vi "Sell Stock.vi"(8 "error in":errorcluster, 10 "quantity":i32=1, 11 "Stock Name":string) -> (0 "error out":errorcluster, 3 "Order":T1)   [LabVIEW 2020, in "Full Featured MCP Server.lvlib"]
doc: "Sells shares of one stock at the current price and returns what was sold: stock, quantity, price per share, total and the wallet afterwards. The order is refused with an error that says why when the name is unknown or you own fewer shares than you want to sell."
uses:
  Full Featured MCP Server.lvlib
  Market/Market Mode.ctl
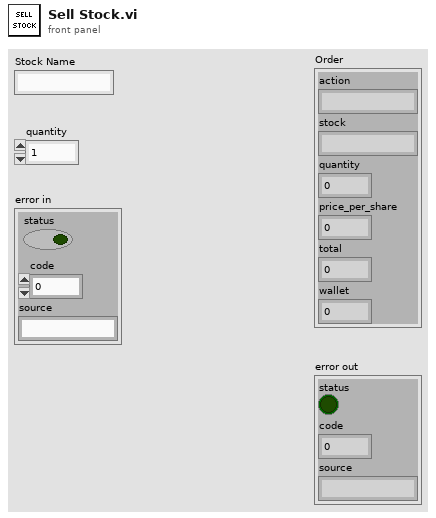
[diagram p1: front panel]
types:
  T1 = cluster{"action":string, "stock":string, "quantity":i32, "price_per_share":dbl, "total":dbl, "wallet":dbl}
  T2 = typedef "Full Featured MCP Server.lvlib/Market Mode.ctl" = enum16{"Get", "Init", "Advance", "Buy", "Sell"}
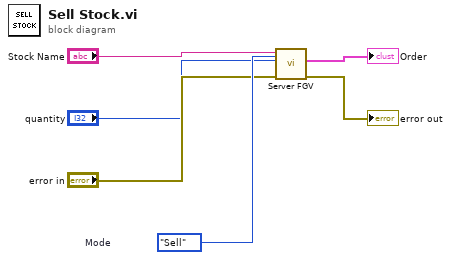
[diagram p0: block diagram]
diagram:
  w4 = Market_Mode."Sell"  # Mode
  n1 = call "Server FGV.vi"("Mode"=w4, "error in"="error in", "quantity"="quantity", "stock name"="Stock Name") -> ("error out"=→"error out":errorcluster, "order"=→"Order":T1)  [unwired: 5 in, 1 out]
